vi "Get Item.vi"(8 "error in (no error)":errorcluster, 11 "in":u32) -> (0 "error out":errorcluster, 3 "OUT":u32)   [LabVIEW 2017, in "HID_ARZ.lvlib"]
doc: "GET_ITEM GetItem;"
uses:
  HID_ARZ.lvlib
  <userlib>/HID_ARZ/mcHID.dll
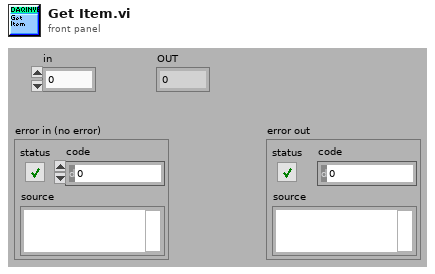
[diagram p1: front panel]
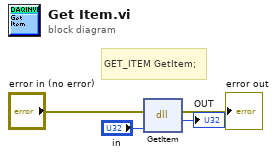
[diagram p0: block diagram]
diagram:
  # "GET_ITEM GetItem;"
  n1 = dll-call lib="C:/Program Files (x86)/National Instruments/LabVIEW 2017/user.lib/HID_ARZ/mcHID.*" fn="GetItem"(error in="error in (no error)", "para0"="in") -> (error out=→"error out":errorcluster, "return type"=→"OUT":u32)  [unwired: 3 in, 1 out]
